vi "ce exmpl - compare 2D arrays.vi"(5 "array for checking":dbl[][](array[numeric]) format="%.2f", 6 "standard array":dbl[][](array[numeric]) format="%.2f") -> (0 "arrays are different":bool, 1 "array sizes are not equal":bool, 2 "max relative difference":T1 {"relative difference, %" format="%#.6g"; "absolute difference" format="%#.6g"}, 3 "max absolute difference":T1 {"relative difference, %" format="%#.6g"; "absolute difference" format="%#.6g"})   [LabVIEW 2021]
doc: "::: CalcExpress Toolkit :::\nCopyright (c) 2000-2026 Konstantin Shifershteyn. All rights reserved."
uses:
  ce exmpl - 2D difference info.ctl
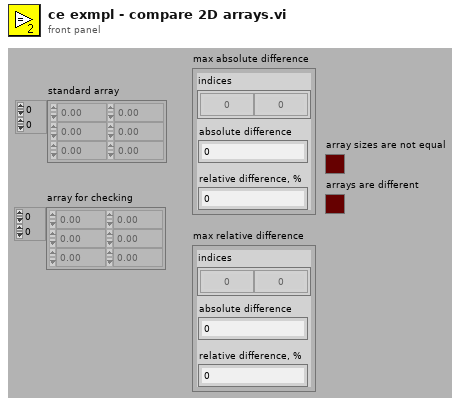
[diagram p1: front panel]
types:
  T1 = typedef "ce exmpl - 2D difference info.ctl" = cluster{"indices":i32[], "absolute difference":dbl, "relative difference, %":dbl}
  T2 = cluster{"indexes":i32[], "absolute difference":dbl, "relative difference, %":dbl}
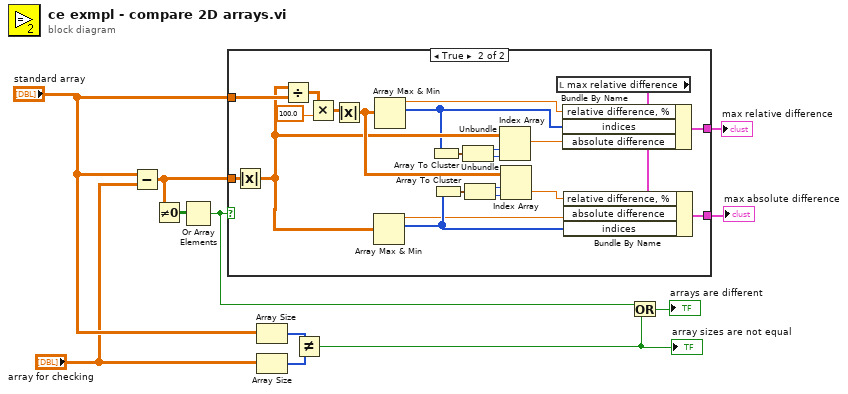
[diagram p0: block diagram]
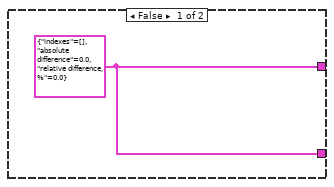
[diagram p2: hidden frame]
diagram:
  n1 = Subtract(x="standard array", y="array for checking") -> (x-y=w5:dbl[][])
  n2 = Not Equal To 0?(x=w5) -> (x != 0?=w7:bool[][])
  n3 = Or Array Elements(Boolean array=w7) -> (logical OR=w1:bool)
  n4 = case shown="True" w1 {
    tunnel: "standard array" -> [_ w30]
    tunnel: [w12 w27] -> w3
    tunnel: [w12 w25] -> w4
    tunnel: w5 -> [_ w23]
    frame False {
      w12 = T2 {"indexes"=[], "absolute difference"=0.0, "relative difference, %"=0.0} ("max relative difference")
    }
    frame True {
      n5 = Absolute Value(x=w23) -> (abs(x)=w22:dbl[][])
      n6 = Divide(x=w22, y=w30) -> (x/y=w33:dbl[][])
      n7 = Multiply(x=w33, y=100.0) -> (x*y=w34:dbl[][])
      n8 = Absolute Value(x=w34) -> (abs(x)=w29:dbl[][])
      n9 = Array Max & Min(array=w22) -> (max value=w14:dbl, max index (indices)=w15:i32[])  [unwired: 2 out]
      n10 = Array Max & Min(array=w29) -> (max value=w24:dbl, max index (indices)=w21:i32[])  [unwired: 2 out]
      n11 = Array To Cluster(array=w21) -> (cluster=w20:cluster{"[0]":i32, "[1]":i32})
      n12 = Array To Cluster(array=w15) -> (cluster=w13:cluster{"[0]":i32, "[1]":i32})
      n13 = Unbundle(w20) -> ("[0]"=w19:i32, "[1]"=w18:i32)
      n14 = Unbundle(w13) -> ("[0]"=w17:i32, "[1]"=w16:i32)
      n15 = Index Array(array=w22, index (row)=w19, index (col)=w18) -> (element=w31:dbl)
      n16 = Index Array(array=w29, index (row)=w17, index (col)=w16) -> (element=w26:dbl)
      n17 = local read "max relative difference"() -> (w28:T1)
      n18 = Bundle By Name(cluster=w28, "relative difference, %"=w24, "indices"=w21, "absolute difference"=w31) -> (w25:T1)
      n19 = Bundle By Name(cluster=w28, "relative difference, %"=w26, "absolute difference"=w14, "indices"=w15) -> (w27:T1)
    }
  }
  "max absolute difference" <- w3
  "max relative difference" <- w4
  n20 = Array Size(array="standard array") -> (size(s)=w11:i32[])
  n21 = Array Size(array="array for checking") -> (size(s)=w10:i32[])
  n22 = Not Equal?(x=w11, y=w10) -> (x != y?=w8:bool)
  "array sizes are not equal" <- w8
  n23 = Or(x=w1, y=w8) -> (x .or. y?=→"arrays are different":bool)
